vi "GetTestDevicePropertyv3.vi"() -> ()   [LabVIEW 2017]
uses:
  <vilib>/httpClient/LabVIEWHTTPClient.lvlib
panel:
  out "data":variant
  out "error out":errorcluster
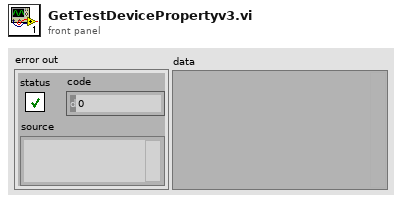
[diagram p1: front panel]
types:
  T1 = typedef "LabVIEWHTTPClient.lvlib/ClientHandle.ctl" = refnum<k1>
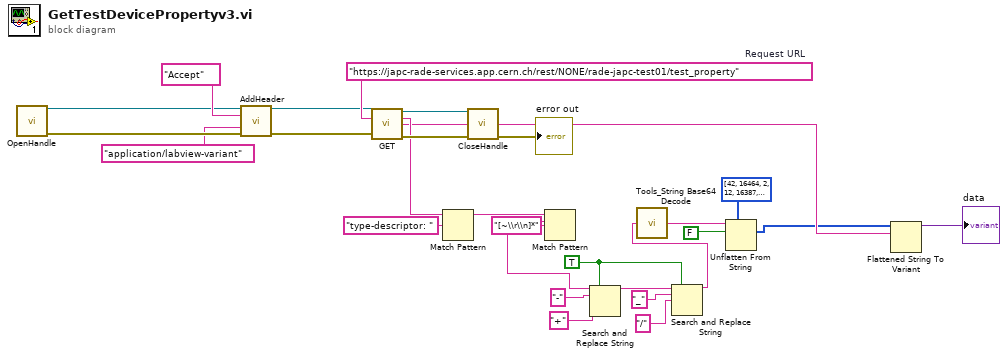
[diagram p0: block diagram]
diagram:
  w8 = TRUE ("replace all? (F)")
  w23 = "https://japc-rade-services.app.cern.ch/rest/NONE/rade-japc-test01/test_property"  # Request URL
  n1 = call <vilib>:"OpenHandle.vi"() -> ("client handle out"=w25:T1, "error out"=w24:errorcluster)  [unwired: 14 in]
  n2 = call <vilib>:"AddHeader.vi"("client handle"=w25, "header"="Accept", "value"="application/labview-variant", "error in (no error)"=w24) -> ("client handle out"=w11:T1, "error out"=w10:errorcluster)  [unwired: 10 in]
  n3 = call <vilib>:"GET.vi"("client handle"=w11, "url"=w23, "error in (no error)"=w10) -> ("client handle out"=w27:T1, "headers"=w20:string, "body"=w16:string, "error out"=w22:errorcluster)  [unwired: 9 in]
  n4 = Match Pattern(string=w20, regular expression="type-descriptor: ") -> (after substring=w18:string)  [unwired: 1 in, 3 out]
  n5 = call <vilib>:"CloseHandle.vi"("client handle"=w27, "error in (no error)"=w22) -> ("error out"=→"error out":errorcluster)  [unwired: 13 in]
  n6 = Match Pattern(string=w18, regular expression="[~\\r\\n]*") -> (match substring=w3:string)  [unwired: 1 in, 3 out]
  n7 = Search and Replace String(replace all?=w8, input string=w3, search string="-" ("replace string (\"\")"), replace string="+" ("substring (\"\")")) -> (result string=w9:string)  [unwired: 4 in, 3 out]
  n8 = Search and Replace String(replace all?=w8, input string=w9, search string="_" ("replace string (\"\")"), replace string="/" ("substring (\"\")")) -> (result string=w2:string)  [unwired: 4 in, 3 out]
  n9 = call <userlib>:"Tools_String Base64 Decode.vi"("Base64 String"=w2) -> ("Normal String"=w1:string)
  n10 = Unflatten From String(type=i16[] [42, 16464, 2, 12, 16387, 1901, 31049, 28276, 13106, 14, 16417, 2413, 31042, 28527, 27749, 24942, 2381, 31059, 25441, 27745, 29299] ("type string"), binary string=w1, data includes array or string size? (T)=FALSE) -> (value=w12:i16[])  [unwired: 2 in, 2 out]
  n11 = Flattened String To Variant(6:w16, 7:w12) -> (3:→"data":variant)  [unwired: 1 in, 1 out]
